vi "Base composit for each signal.vi"(8 "文字列":string, 11 "Base Composition":string[](array[string])) -> (3 "Base C":i32[](array[numeric]))   [LabVIEW 2018]
panel:
  out "サイズ":i32[](array[numeric])
  out "配列 2":bool[][](array[boolean])
  out "配列":bool[](array[boolean])
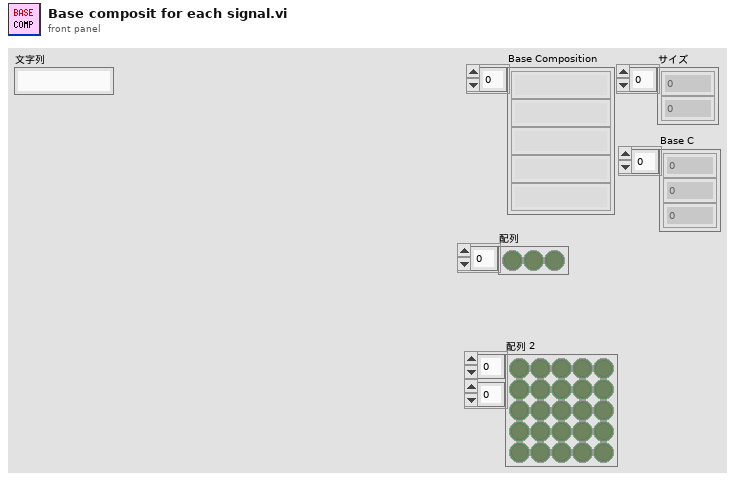
[diagram p1: front panel]
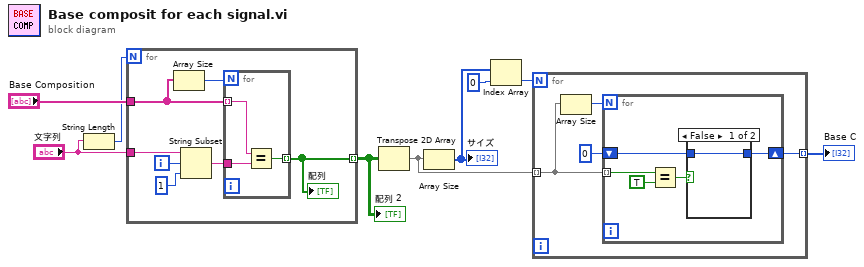
[diagram p0: block diagram]
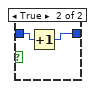
[diagram p2: hidden frame]
diagram:
  n1 = String Length(string="文字列") -> (length=w7:i32)
  n2 = for {
    N: w7 -> [_]
    tunnel: "Base Composition" -> [w11]
    tunnel: "文字列" -> [w14]
    tunnel: [w12] -> w6 mode=indexing
    i -> [w16]
    n3 = Array Size(array=w11) -> (size(s)=w10:i32)
    n4 = String Subset(string=w14, offset (0)=w16, length (rest)=1 ("長さ（残り）")) -> (substring=w13:string)
    n5 = for {
      N: w10 -> [_]
      tunnel: w13 -> [w18]
      tunnel: w11 -> [w19] mode=indexing
      tunnel: [w17] -> w12 mode=indexing
      n6 = Equal?(x=w19, y=w18) -> (x = y?=w17:bool)
    }
    "配列" <- w12
  }
  "配列 2" <- w6
  n7 = Transpose 2D Array(2D array=w6) -> (transposed array=w2:bool[][])
  n8 = Array Size(array=w2) -> (size(s)=w3:i32[])
  "サイズ" <- w3
  n9 = Index Array(array=w3, index=0 ("指標")) -> (element=w4:i32)
  n10 = for {
    N: w4 -> [_]
    tunnel: w2 -> [w22] mode=indexing
    tunnel: [w20] -> w1 mode=indexing
    n11 = Array Size(array=w22) -> (size(s)=w23:i32)
    n12 = for {
      N: w23 -> [_]
      tunnel: w22 -> [w28] mode=indexing
      shift-right: [w25] -> w20
      shift-left: 0 -> [w24]
      n13 = Equal?(x=w28, y=TRUE) -> (x = y?=w26:bool)
      n14 = case shown="False" w26 {
        tunnel: [w29 w31] -> w25
        tunnel: w24 -> [w29 w30]
        frame False {
        }
        frame True {
          n15 = Increment(x=w30) -> (x+1=w31:i32)
        }
      }
    }
  }
  "Base C" <- w1
